vi "Func - Error Status to Error Cluster.vi"(9 "error status in":bool) -> (0 "Error Cluster out":errorcluster, 1 "error status out":bool)   [LabVIEW 2021]
doc: "This VI converts a Boolean error status to the standard error cluster. Refer to the VI help for more details.\n\n::: CalcExpress Toolkit :::\nCopyright (c) 2000-2026 Konstantin Shifershteyn. All rights reserved."
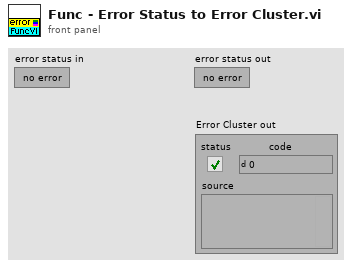
[diagram p1: front panel]
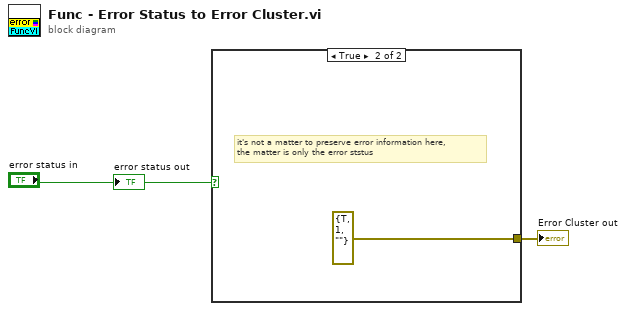
[diagram p0: block diagram]
diagram:
  n1 = case shown="True" "error status in" {
    tunnel: [_ errorcluster {"status"=TRUE, "code"=1, "source"=""} ("error constant")] -> w2
    frame False {
    }
    frame True {
      # "it's not a matter to preserve error information here,\nthe matter is only the error ststus"
    }
  }
  "Error Cluster out" <- w2
  "error status out" <- "error status in"
